vi "FuncVI-sfmake.vi"(5 "InstanceRef":T2, 9 "arg list":T1[](array[typedef]) {"num" format="%.2f"}) -> (0 "error out":bool, 3 "result":T1 {"num" format="%.2f"})   [LabVIEW 2021]
doc: "::: CalcExpress Toolkit :::\nCopyright (c) 2000-2026 Konstantin Shifershteyn. All rights reserved."
uses:
  cetypes.llb/CalcExpress Function Argument Info.ctl
  cetypes.llb/CalcExpress Instance RefNum.ctl
panel:
  in  "max arg num":i32=2
  in  "min arg num":i32=2
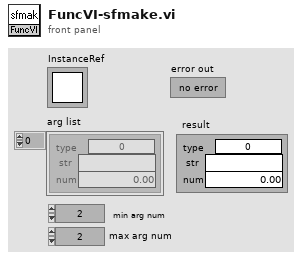
[diagram p1: front panel]
types:
  T1 = typedef "CalcExpress Function Argument Info.ctl" = cluster{"type":u32, "str":string, "num":dbl}
  T2 = typedef "CalcExpress Instance RefNum.ctl" = refnum<k1>
  T3 = cluster{"index":i32, "data type":enum32{"String", "DBL Number", "identifier", "1D Array of DBL", "2D Array of DBL", "CDB Number", "1D Array of CDB", "2D Array of CDB", "1D Array of String", "2D Array of String", "Unknown data type"}, "default num":dbl, "default str":string}
  T4 = enum32{"String", "DBL Number", "identifier", "1D Array of DBL", "2D Array of DBL", "CDB Number", "1D Array of CDB", "2D Array of CDB", "1D Array of String", "2D Array of String", "Unknown data type"}
  T5 = cluster{"index":i32, "any type":i32, "default num":dbl, "default str":string}
  T6 = cluster{"index":i32, "any type":u32, "default num":dbl, "default str":string}[]
  T7 = cluster{"data type":enum32{"String", "DBL Number", "identifier", "1D Array of DBL", "2D Array of DBL", "CDB Number", "1D Array of CDB", "2D Array of CDB", "1D Array of String", "2D Array of String", "Unknown data type"}, "data string":string, dbl}
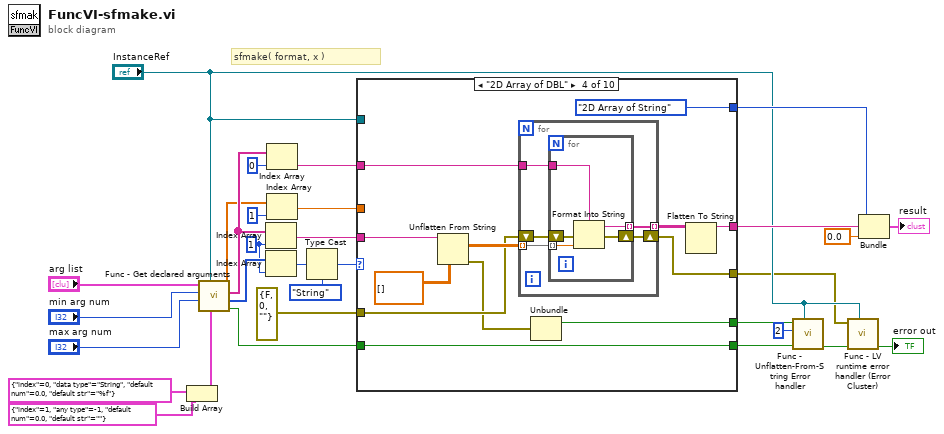
[diagram p0: block diagram]
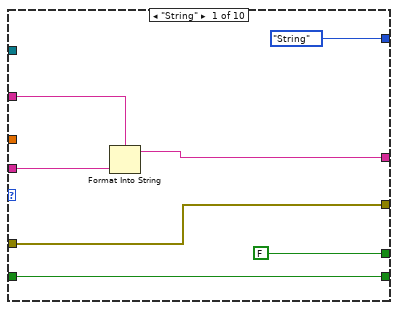
[diagram p2: hidden frame]
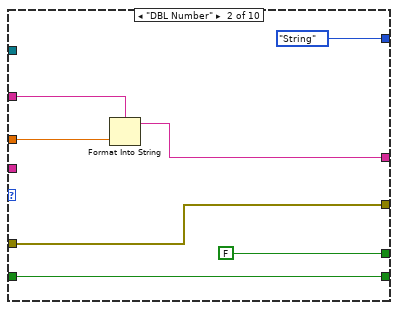
[diagram p3: hidden frame]
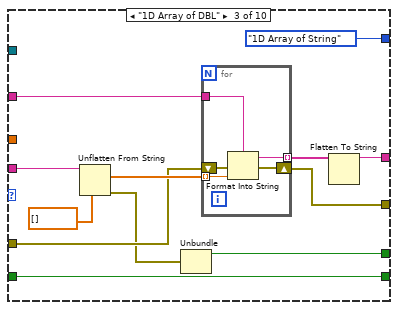
[diagram p4: hidden frame]
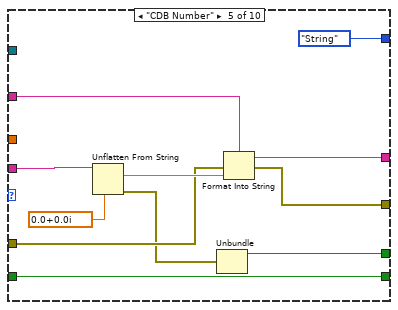
[diagram p5: hidden frame]
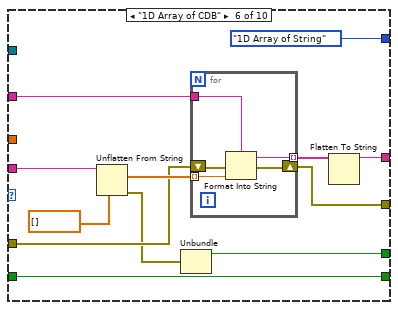
[diagram p6: hidden frame]
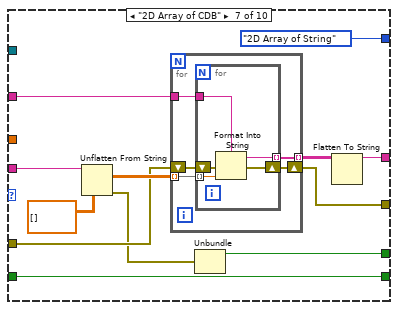
[diagram p7: hidden frame]
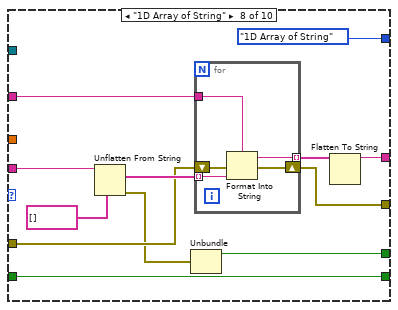
[diagram p8: hidden frame]
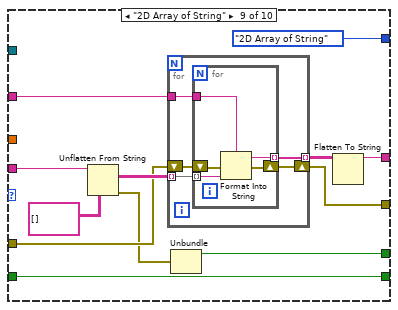
[diagram p9: hidden frame]
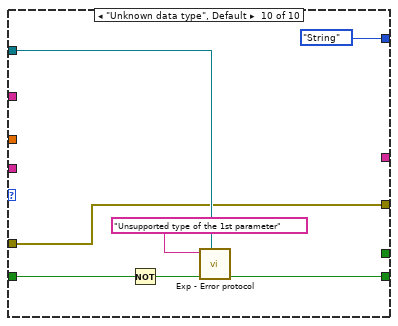
[diagram p10: hidden frame]
diagram:
  w19 = 1
  # "sfmake( format, x )"
  n1 = Build Array(T3 {"index"=0, "data type"=enum."String", "default num"=0.0, "default str"="%f"} ("arg descriptor"), T5 {"index"=1, "any type"=-1, "default num"=0.0, "default str"=""} ("arg descriptor")) -> (w26:T6)
  n2 = call "Func - Get declared arguments.vi"("arg descriptors"=w26, "InstanceRef"="InstanceRef", "max arg num"="max arg num", "min arg num"="min arg num", "arg list"="arg list") -> ("error out"=w18:bool, "type list"=w21:u32[], "str list"=w20:string[], "num list"=w17:dbl[])  [unwired: 3 in]
  n3 = Index Array(array=w20, index=w19) -> (element=w22:string)
  n4 = Index Array(array=w21, index=w19) -> (element=w23:u32)
  n5 = Index Array(array=w20, index=0) -> (element=w28:string)
  n6 = Index Array(array=w17, index=1) -> (element=w29:dbl)
  n7 = Type Cast(type=T4."String" ("data type"), x=w23) -> (*(type *) &x=w24:T4)
  n8 = case shown="\"2D Array of DBL\"" w24 {
    tunnel: w22 -> [w34 _ w57 w74 w91 w107 w124 w146 w163 _]
    tunnel: w29 -> [_ w42 _ _ _ _ _ _ _ _]
    tunnel: w28 -> [w37 w44 w53 w70 w94 w103 w120 w142 w159 _]
    tunnel: w18 -> [w38 w45 w55 w72 w95 w105 w122 w144 w161 w180]
    tunnel: [w38 w45 w55 w72 w95 w105 w122 w144 w161 w178] -> w10
    tunnel: "InstanceRef" -> [_ _ _ _ _ _ _ _ _ w177]
    tunnel: [w35 w41 w51 w68 w92 w101 w118 w140 w157 _] -> w16
    tunnel: [T4."String" ("data type") T4."String" ("data type") T4."1D Array of String" ("data type") T4."2D Array of String" ("data type") T4."String" ("data type") T4."1D Array of String" ("data type") T4."2D Array of String" ("data type") T4."1D Array of String" ("data type") T4."2D Array of String" ("data type") T4."String" ("data type")] -> w14
    tunnel: [FALSE ("err") FALSE ("err") w49 w64 w87 w97 w116 w137 w153 _] -> w9
    tunnel: [w33 w39 w47 w66 w88 w98 w115 w136 w154 w174] -> w1
    tunnel: errorcluster {"status"=FALSE, "code"=0, "source"=""} ("error IO") -> [w33 w39 w48 w65 w86 w99 w114 w138 w155 w174]
    frame "String" {
      n9 = Format Into String(format string=w37, w34) -> (resulting string=w35:string)  [unwired: 2 in, 1 out]
    }
    frame "DBL Number" {
      n10 = Format Into String(format string=w44, w42) -> (resulting string=w41:string)  [unwired: 2 in, 1 out]
    }
    frame "1D Array of DBL" {
      n11 = Unflatten From String(type=dbl[] [], binary string=w57) -> (value=w54:dbl[], error out=w46:errorcluster)  [unwired: 3 in, 1 out]
      n12 = Unbundle(w46) -> ("status"=w49:bool)  [unwired: 2 out]
      n13 = for {
        tunnel: w54 -> [w62] mode=indexing
        tunnel: w53 -> [w61]
        tunnel: [w60] -> w52 mode=indexing
        shift-right: [w59] -> w47
        shift-left: w48 -> [w58]
        n14 = Format Into String(format string=w61, error in=w58, w62) -> (resulting string=w60:string, error out=w59:errorcluster)  [unwired: 1 in]
      }
      n15 = Flatten To String(anything=w52) -> (data string=w51:string)  [unwired: 3 in, 2 out]
    }
    frame "2D Array of DBL" {
      n16 = Unflatten From String(type=dbl[][] [], binary string=w74) -> (value=w71:dbl[][], error out=w63:errorcluster)  [unwired: 3 in, 1 out]
      n17 = for {
        tunnel: w71 -> [w79] mode=indexing
        tunnel: w70 -> [w78]
        tunnel: [w77] -> w69 mode=indexing
        shift-right: [w75] -> w66
        shift-left: w65 -> [w76]
        n18 = for {
          tunnel: w79 -> [w84] mode=indexing
          tunnel: w78 -> [w83]
          tunnel: [w82] -> w77 mode=indexing
          shift-right: [w80] -> w75
          shift-left: w76 -> [w81]
          n19 = Format Into String(format string=w83, error in=w81, w84) -> (resulting string=w82:string, error out=w80:errorcluster)  [unwired: 1 in]
        }
      }
      n20 = Unbundle(w63) -> ("status"=w64:bool)  [unwired: 2 out]
      n21 = Flatten To String(anything=w69) -> (data string=w68:string)  [unwired: 3 in, 2 out]
    }
    frame "CDB Number" {
      n22 = Unflatten From String(type=cdb 0.0+0.0i, binary string=w91) -> (value=w89:cdb, error out=w85:errorcluster)  [unwired: 3 in, 1 out]
      n23 = Unbundle(w85) -> ("status"=w87:bool)  [unwired: 2 out]
      n24 = Format Into String(format string=w94, error in=w86, w89) -> (resulting string=w92:string, error out=w88:errorcluster)  [unwired: 1 in]
    }
    frame "1D Array of CDB" {
      n25 = Unflatten From String(type=cdb[] [], binary string=w107) -> (value=w104:cdb[], error out=w96:errorcluster)  [unwired: 3 in, 1 out]
      n26 = Unbundle(w96) -> ("status"=w97:bool)  [unwired: 2 out]
      n27 = for {
        tunnel: w104 -> [w112] mode=indexing
        tunnel: w103 -> [w111]
        tunnel: [w110] -> w102 mode=indexing
        shift-right: [w109] -> w98
        shift-left: w99 -> [w108]
        n28 = Format Into String(format string=w111, error in=w108, w112) -> (resulting string=w110:string, error out=w109:errorcluster)  [unwired: 1 in]
      }
      n29 = Flatten To String(anything=w102) -> (data string=w101:string)  [unwired: 3 in, 2 out]
    }
    frame "2D Array of CDB" {
      n30 = Unflatten From String(type=cdb[][] [], binary string=w124) -> (value=w121:cdb[][], error out=w113:errorcluster)  [unwired: 3 in, 1 out]
      n31 = for {
        tunnel: w121 -> [w129] mode=indexing
        tunnel: w120 -> [w128]
        tunnel: [w127] -> w119 mode=indexing
        shift-right: [w126] -> w115
        shift-left: w114 -> [w125]
        n32 = for {
          tunnel: w129 -> [w134] mode=indexing
          tunnel: w128 -> [w133]
          tunnel: [w132] -> w127 mode=indexing
          shift-right: [w131] -> w126
          shift-left: w125 -> [w130]
          n33 = Format Into String(format string=w133, error in=w130, w134) -> (resulting string=w132:string, error out=w131:errorcluster)  [unwired: 1 in]
        }
      }
      n34 = Unbundle(w113) -> ("status"=w116:bool)  [unwired: 2 out]
      n35 = Flatten To String(anything=w119) -> (data string=w118:string)  [unwired: 3 in, 2 out]
    }
    frame "1D Array of String" {
      n36 = Unflatten From String(type=string[] [], binary string=w146) -> (value=w143:string[], error out=w135:errorcluster)  [unwired: 3 in, 1 out]
      n37 = Unbundle(w135) -> ("status"=w137:bool)  [unwired: 2 out]
      n38 = for {
        tunnel: w143 -> [w151] mode=indexing
        tunnel: w142 -> [w150]
        tunnel: [w149] -> w141 mode=indexing
        shift-right: [w148] -> w136
        shift-left: w138 -> [w147]
        n39 = Format Into String(format string=w150, error in=w147, w151) -> (resulting string=w149:string, error out=w148:errorcluster)  [unwired: 1 in]
      }
      n40 = Flatten To String(anything=w141) -> (data string=w140:string)  [unwired: 3 in, 2 out]
    }
    frame "2D Array of String" {
      n41 = Unflatten From String(type=string[][] [], binary string=w163) -> (value=w160:string[][], error out=w152:errorcluster)  [unwired: 3 in, 1 out]
      n42 = for {
        tunnel: w160 -> [w168] mode=indexing
        tunnel: w159 -> [w167]
        tunnel: [w166] -> w158 mode=indexing
        shift-right: [w164] -> w154
        shift-left: w155 -> [w165]
        n43 = for {
          tunnel: w168 -> [w173] mode=indexing
          tunnel: w167 -> [w172]
          tunnel: [w171] -> w166 mode=indexing
          shift-right: [w169] -> w164
          shift-left: w165 -> [w170]
          n44 = Format Into String(format string=w172, error in=w170, w173) -> (resulting string=w171:string, error out=w169:errorcluster)  [unwired: 1 in]
        }
      }
      n45 = Unbundle(w152) -> ("status"=w153:bool)  [unwired: 2 out]
      n46 = Flatten To String(anything=w158) -> (data string=w157:string)  [unwired: 3 in, 2 out]
    }
    frame "Unknown data type", Default {
      n47 = Not(x=w180) -> (.not. x?=w179:bool)
      n48 = call "Exp - Error protocol.vi"("InstanceRef"=w177, "error in"=w179, "error message in"="Unsupported type of the 1st parameter" ("ErrStr")) -> ("error out"=w178:bool)  [unwired: 5 in, 1 out]
    }
  }
  n49 = call "Func - Unflatten-From-String Error handler.vi"("InstanceRef"="InstanceRef", "error in"=w10, "argument number"=2, "Unflatten Error status"=w9) -> ("error out"=w4:bool)  [unwired: 5 in]
  n50 = call "Func - LV runtime error handler (Error Cluster).vi"("InstanceRef"="InstanceRef", "error in"=w4, "LabVIEW error"=w1) -> ("error out"=→"error out":bool)  [unwired: 3 in, 3 out]
  n51 = Bundle("data type"=w14, "data string"=w16, 0.0) -> (→"result":T7)  [unwired: 1 in]
